vi "Task Type.vi"(8 "error in (no error)":errorcluster, 11 "Task in":refnum<class "Task Config.lvclass">) -> (0 "error out":errorcluster, 2 "Task Type":string, 3 "Task out":refnum<class "Task Config.lvclass">)   [LabVIEW 2020, in "VolatusConfig.lvlib" / "Task Config.lvclass"]
uses:
  Task Config.lvclass
  C:/dev/lv20CE/relink/lv-volatus/VolatusConfig/VolatusConfigElement/VolatusConfigElement.lvclass
  Meta Name.ctl
  VolatusConfigElement/VolatusConfigElement.lvclass/VolatusConfigElement.ctl
  Task Config.lvclass/Task Config.ctl
  lv-cdm/CDM-Config/Config Element/Config Element.lvclass
  VolatusConfig.lvlib
  VolatusConfigElement/VolatusConfigElement.lvclass
  C:/dev/lv20CE/relink/lv-volatus/VolatusConfig/Task/Task Config.lvclass
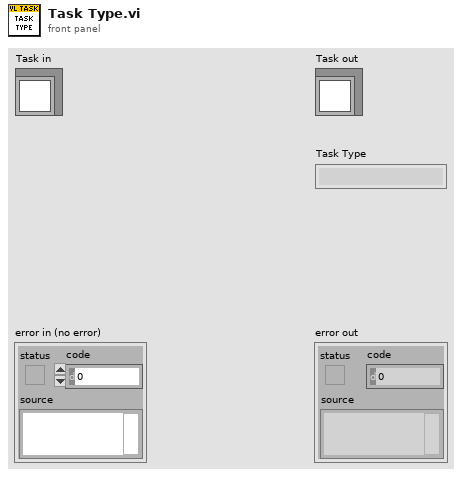
[diagram p1: front panel]
types:
  T1 = typedef "VolatusConfig.lvlib/Meta Name.ctl" = enum16{"VL_Type", "VL_Node_IP", "VL_Node_Type", "VL_Task_Type", "VL_Group_Type", "VL_Channel_Type", "VL_Channel_DataType", "VL_Config_Version", "VL_Overlay_Type", "VL_Config_Hash"}
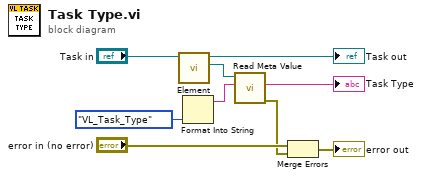
[diagram p0: block diagram]
diagram:
  n1 = call "Element.vi"("VolatusConfigElement in"="Task in") -> ("Element"=w1:refnum<class "Config Element.lvclass">, "VolatusConfigElement out"=→"Task out":refnum<class "Task Config.lvclass">)  [unwired: 9 in]
  n2 = Format Into String(Meta_Name."VL_Task_Type" ("Meta Name")) -> (resulting string=w6:string)  [unwired: 3 in, 1 out]
  n3 = call "Read Meta Value.vi"("Meta Name"=w6, "Config Element in"=w1) -> ("error out"=w3:errorcluster, "Meta Value"=→"Task Type":string)  [unwired: 7 in, 1 out]
  n4 = Merge Errors("error in (no error)", w3) -> (→"error out":errorcluster)
